vi "RDC-Array-calc_propagation_const.vi"(7 "dielectric":T1, 10 "Measured open":T2, 11 "Measured Short":T2) -> (1 "calc prop const mix 2":cdb[](array[numeric]), 2 "e gamma mix":cdb[](array[numeric]))   [LabVIEW 2020, in "RDC-Reflection_Data_Computation.lvlib"]
doc: "Combines the measurement-based and formula-based propagation constants from a measured open and short Common Format cluster and the selected coax dielectric. Returns the mixed propagation constant and the e gamma mix array used by RDC-Array-Reflection_Correction."
uses:
  RDC-Reflection_Data_Computation.lvlib
  Reflector/RFH-common_data_format.ctl
  RDC-dielectric_types.ctl
  Reflector/RFH-Reflection_File_Handler.lvlib
panel:
  out "tau 2":dbl format="%#_6p"
  out "tau":dbl format="%#_6p"
  out "beta":dbl[][](graph)
  out "Alpha":dbl[][](graph)
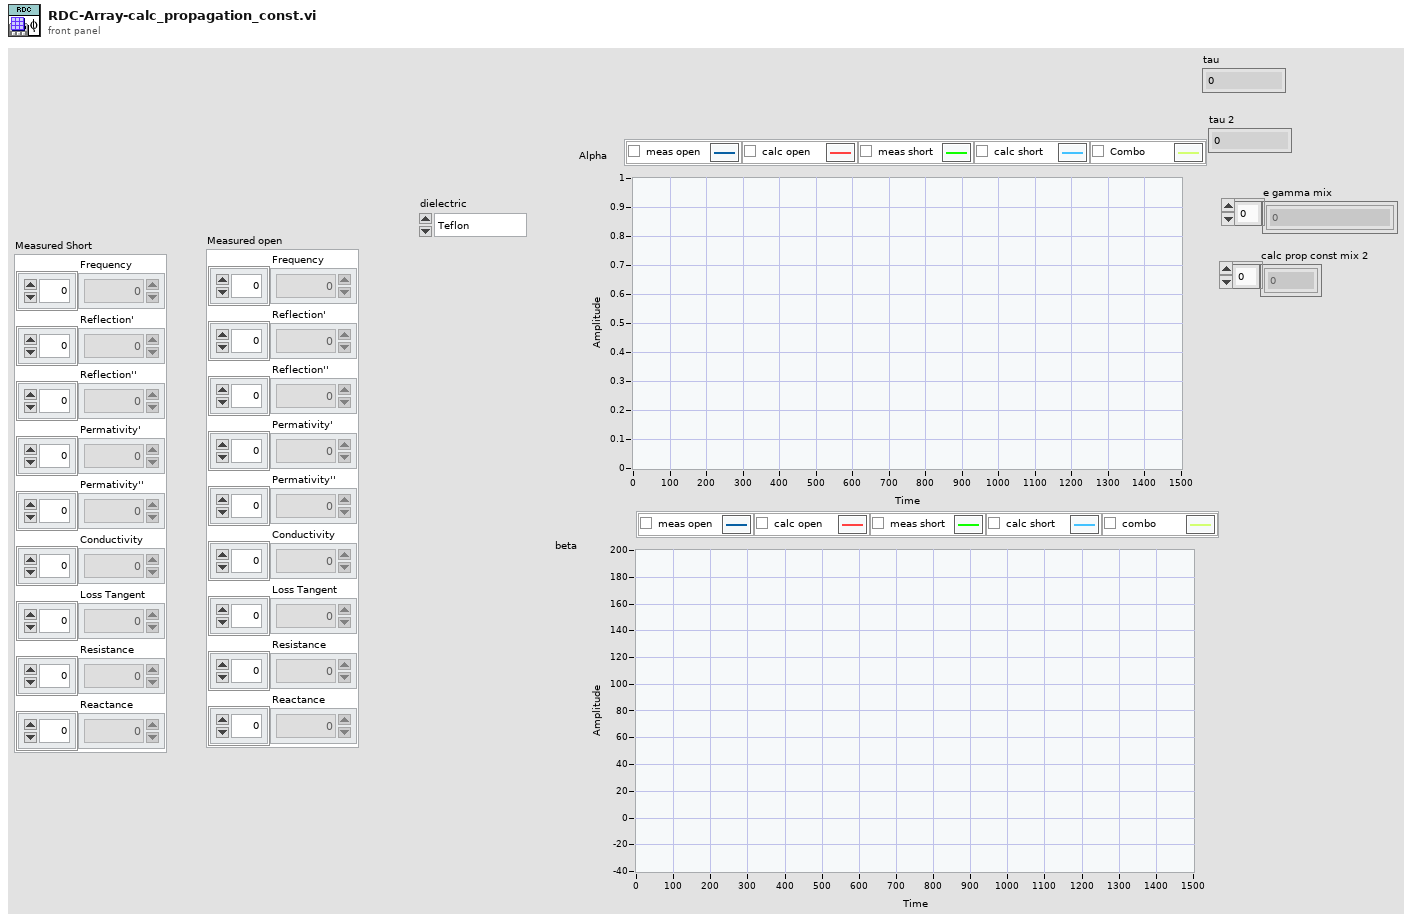
[diagram p1: front panel]
types:
  T1 = typedef "RDC-Reflection_Data_Computation.lvlib/RDC-dielectric_types.ctl" = enum16{"Teflon", "Eccostock 0005"}
  T2 = typedef "RFH-Reflection_File_Handler.lvlib/RFH-common_data_format.ctl" = cluster{"Frequency":dbl[], "Reflection'":dbl[], "Reflection''":dbl[], "Permativity'":dbl[], "Permativity''":dbl[], "Conductivity":dbl[], "Loss Tangent":dbl[], "Resistance":dbl[], "Reactance":dbl[]}
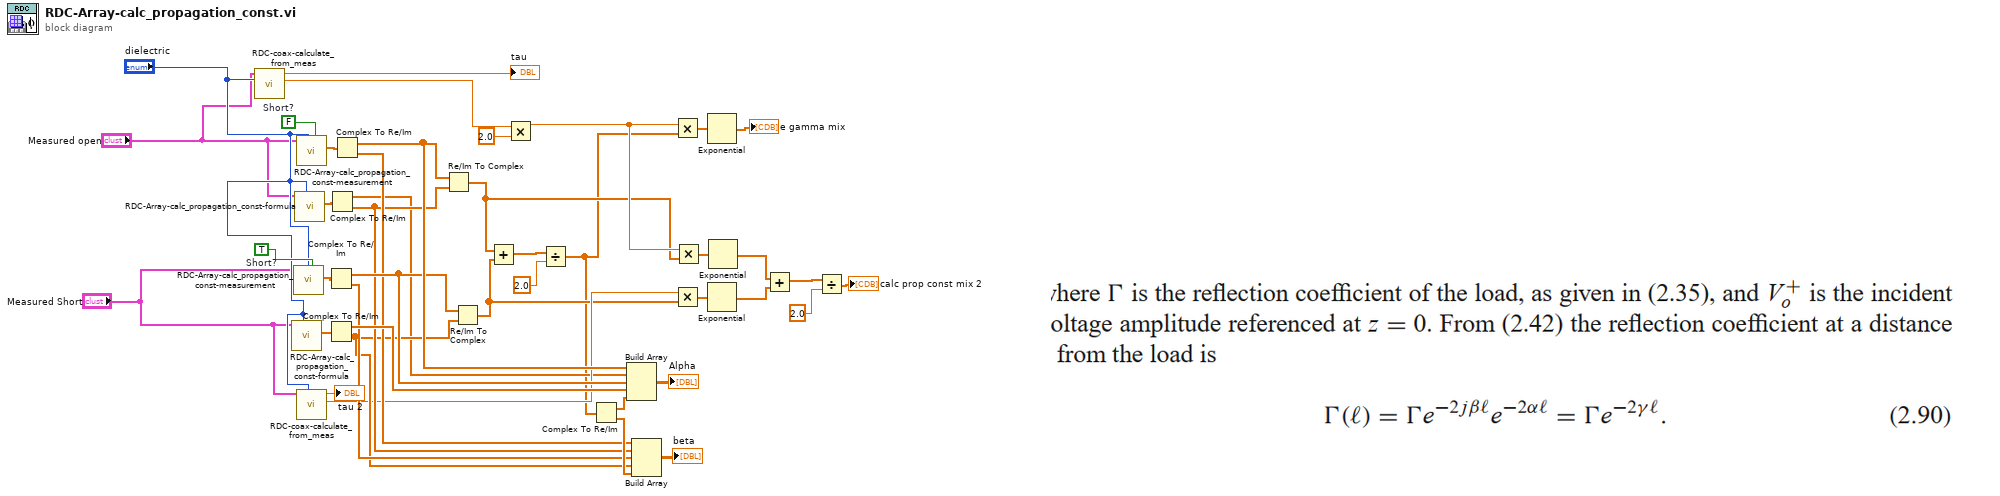
[diagram p0: block diagram]
diagram:
  w38 = TRUE  # Short?
  w39 = FALSE  # Short?
  n1 = call "RDC-coax-calculate_from_meas.vi"("dielectric"="dielectric", "measurement"="Measured open") -> ("lenght [m]"=w9:dbl, "tau"=→"tau":dbl)  [unwired: 7 in, 1 out]
  n2 = call "RDC-Array-calc_propagation_const-formula.vi"("dielectric"="dielectric", "Measured"="Measured Short") -> ("calc prop const"=w34:cdb[])  [unwired: 9 in]
  n3 = call "RDC-Array-calc_propagation_const-measurement.vi"("Short?"=w38, "dielectric"="dielectric", "Measured"="Measured Short") -> ("calc prop const"=w35:cdb[])  [unwired: 8 in]
  n4 = call "RDC-Array-calc_propagation_const-formula.vi"("dielectric"="dielectric", "Measured"="Measured open") -> ("calc prop const"=w36:cdb[])  [unwired: 9 in]
  n5 = call "RDC-Array-calc_propagation_const-measurement.vi"("Short?"=w39, "dielectric"="dielectric", "Measured"="Measured open") -> ("calc prop const"=w37:cdb[])  [unwired: 8 in]
  n6 = call "RDC-coax-calculate_from_meas.vi"("dielectric"="dielectric", "measurement"="Measured Short") -> ("lenght [m]"=w6:dbl, "tau"=→"tau 2":dbl)  [unwired: 7 in, 1 out]
  n7 = Complex To Re/Im(x + iy=w35) -> (x=w29:dbl[], y=w22:dbl[])
  n8 = Complex To Re/Im(x + iy=w34) -> (x=w28:dbl[], y=w21:dbl[])
  n9 = Complex To Re/Im(x + iy=w36) -> (x=w3:dbl[], y=w23:dbl[])
  n10 = Complex To Re/Im(x + iy=w37) -> (x=w30:dbl[], y=w24:dbl[])
  n11 = Re/Im To Complex(1:w23, 2:w30) -> (0:w12:cdb[])
  n12 = Re/Im To Complex(1:w21, 2:w29) -> (0:w2:cdb[])
  n13 = Add(x=w12, y=w2) -> (x+y=w41:cdb[])
  n14 = Multiply(x=w9, y=2.0) -> (x*y=w13:dbl)
  n15 = Divide(x=w41, y=2.0 ("x")) -> (x/y=w1:cdb[])
  n16 = Complex To Re/Im(x + iy=w1) -> (x=w27:dbl[], y=w25:dbl[])
  n17 = Build Array(w30, w3, w29, w28, w27) -> (→"Alpha":dbl[][])
  n18 = Build Array(w24, w23, w22, w21, w25) -> (→"beta":dbl[][])
  n19 = Multiply(x=w13, y=w1) -> (x*y=w32:cdb[])
  n20 = Multiply(x=w6, y=w2) -> (x*y=w18:cdb[])
  n21 = Multiply(x=w13, y=w12) -> (x*y=w19:cdb[])
  n22 = Exponential(1:w32) -> (0:→"e gamma mix":cdb[])
  n23 = Exponential(1:w18) -> (0:w14:cdb[])
  n24 = Exponential(1:w19) -> (0:w15:cdb[])
  n25 = Add(x=w15, y=w14) -> (x+y=w16:cdb[])
  n26 = Divide(x=w16, y=2.0 ("x")) -> (x/y=→"calc prop const mix 2":cdb[])
